vi "IDS Set Get Parameter.vi"(0 "IDS Notifier":refnum<notifier>, 5 "IDS Actions":T1, 7 "IDS Camera Ref":refnum<k24>, 11 "Error":errorcluster) -> (4 "IDS Notifier":refnum<notifier>, 15 "Error":errorcluster)   [LabVIEW 2021]
uses:
  IDS Controls/IDS Notifier Element.ctl
  IDS Controls/IDS Actions.ctl
  IDS Controls/IDS Parameters.ctl
  IDS Controls/IDS Parameter List.ctl
  IDS Controls/IDS ROI.ctl
  <vilib>/vision/Image Controls.llb/IMAQ Image.ctl
  C:/Users/Ries Lab/Documents/Microscope Control from Sheng Account/Microscope-Control/Device Library/Cameras/IDS/IDS LabView Examples/LabVIEW/ueye.NET/uEyeDotNet.dll
  IDS LabView Examples/LabVIEW/ueye.NET/uEyeDotNet.dll
panel:
  out "s32FactorNew":i32
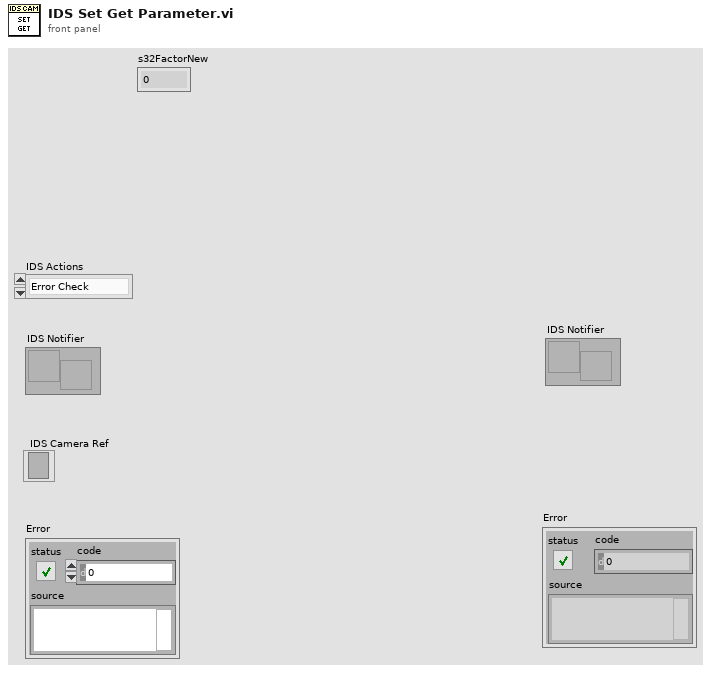
[diagram p1: front panel]
types:
  T1 = typedef "IDS Actions.ctl" = enum16{"Error Check", "Initialize", "Preview", "Record", "Abort", "Record Settings", "Set Parameter", "Get Parameter", "Set ROI", "Get ROI", "Status", "Quit"}
  T2 = typedef "IDS Notifier Element.ctl" = cluster{"IDS Actions":T1, "Received?":bool, "IDS Parameter":T3, "IDS ROI":T5, "Running?":bool, "File Path":path, "# of frames":u32, "Image Ref":T6, "Error":errorcluster, "Binning":i32}
  T3 = typedef "IDS Parameters.ctl" = cluster{"Parameter":T4, "Value":dbl}
  T4 = typedef "IDS Parameter List.ctl" = enum16{"Exposure Time (s)", "Binning", "Gain", "Gamma"}
  T5 = typedef "IDS ROI.ctl" = cluster{"H Offset":i32, "V Offset":i32, "H Width":i32, "V Width":i32}
  T6 = typedef "IMAQ Image.ctl" = refnum<image>
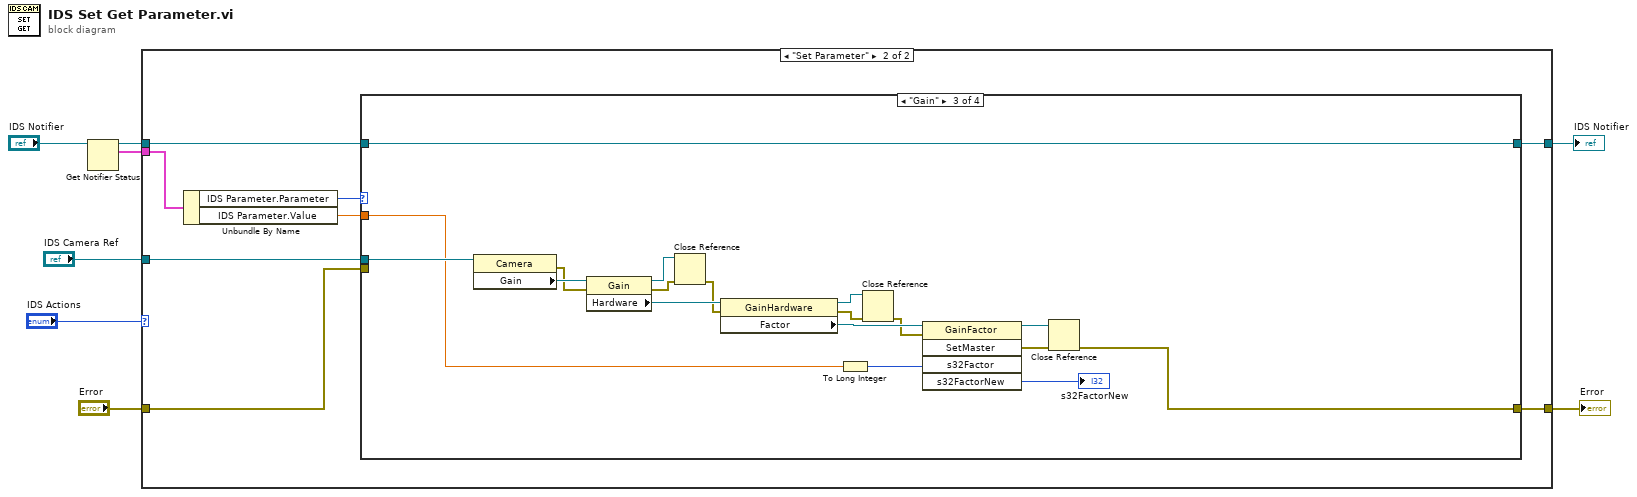
[diagram p0: block diagram]
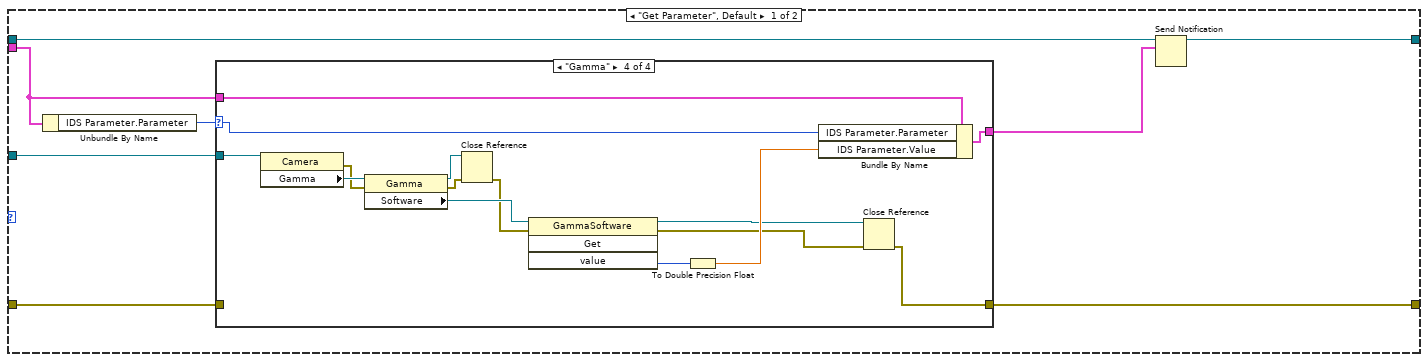
[diagram p2: hidden frame]
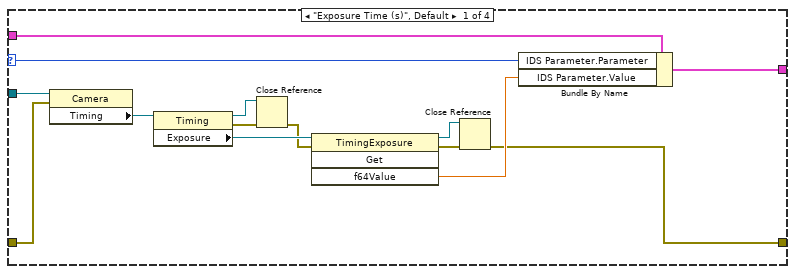
[diagram p3: hidden frame]
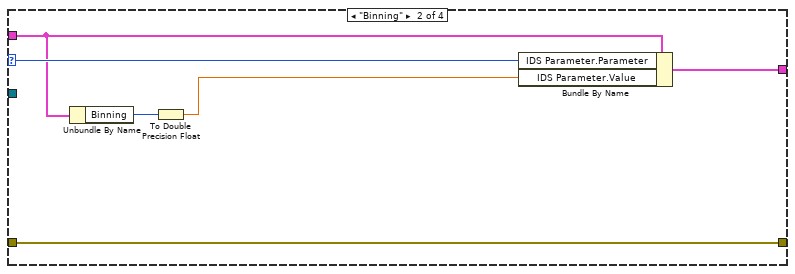
[diagram p4: hidden frame]
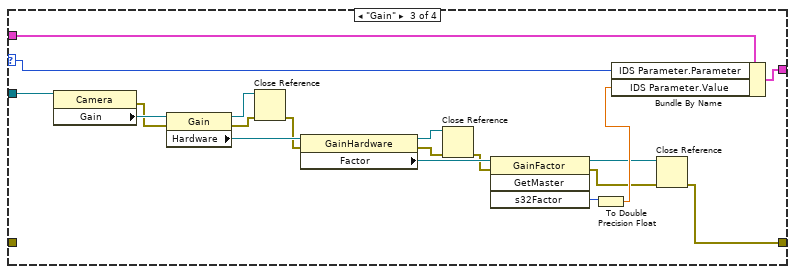
[diagram p5: hidden frame]
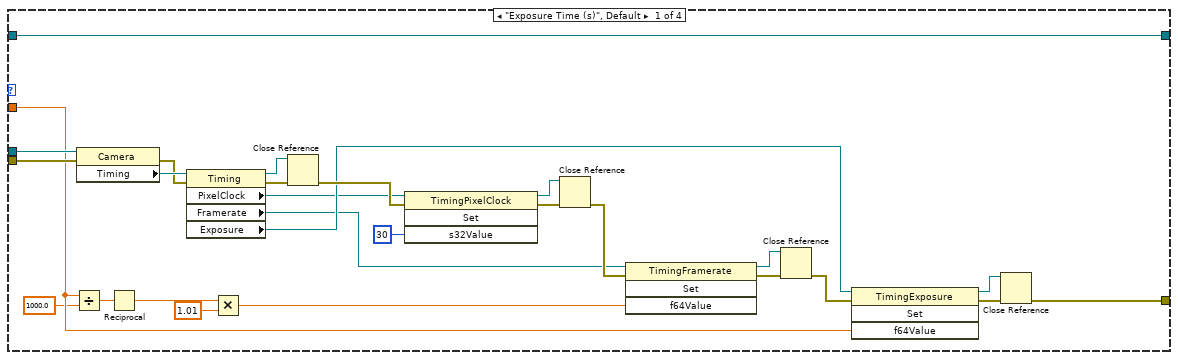
[diagram p6: hidden frame]
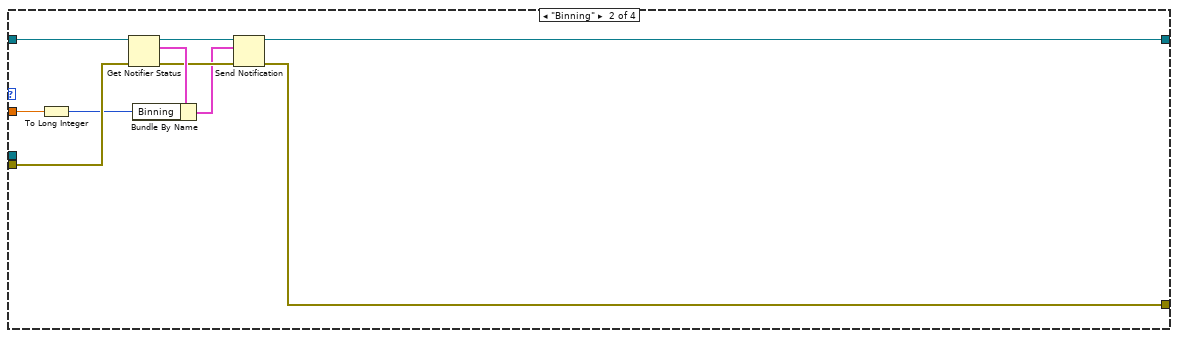
[diagram p7: hidden frame]
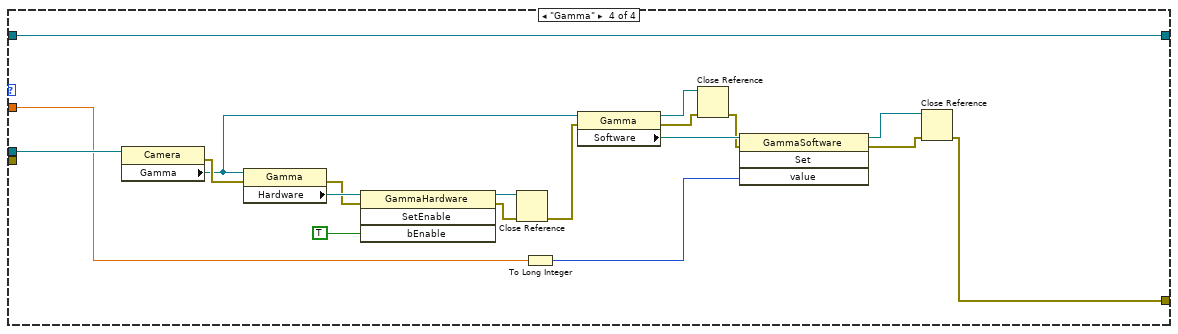
[diagram p8: hidden frame]
diagram:
  n1 = Get Notifier Status(notifier="IDS Notifier") -> (notifier out=w6:refnum<notifier>, current notification=w5:T2)  [unwired: 1 in, 3 out]
  n2 = case shown="\"Set Parameter\"" "IDS Actions" {
    tunnel: w6 -> [w11 w72]
    tunnel: w5 -> [w12 w78]
    tunnel: [w10 w71] -> w3
    tunnel: "IDS Camera Ref" -> [w13 w75]
    tunnel: "Error" -> [w15 w74]
    tunnel: [w14 w73] -> w1
    frame "Get Parameter", Default {
      n3 = Unbundle By Name(w12) -> ("IDS Parameter.Parameter"=w16:T4)
      n4 = case shown="\"Gamma\"" w16 {
        selector: w16 -> [w21 w36 w42 w63]
        tunnel: w15 -> [w18 w33 _ _]
        tunnel: [w17 w33 w37 w58] -> w14
        tunnel: w13 -> [w30 _ w45 w66]
        tunnel: w12 -> [w22 w34 w44 w65]
        tunnel: [w19 w35 w43 w64] -> w9
        frame "Exposure Time (s)", Default {
          n5 = property class="Camera"(reference=w30, error in=w18) -> ("Timing"=w29:refnum<k24>)  [unwired: 2 out]
          n6 = property class="Timing"(reference=w29) -> (reference out=w27:refnum<k24>, error out=w26:errorcluster, "Exposure"=w28:refnum<k24>)  [unwired: 1 in]
          n7 = Close Reference(reference=w27, error in (no error)=w26) -> (error out=w25:errorcluster)
          n8 = invoke class="TimingExposure" method="Get"(reference=w28, error in=w25) -> (reference out=w24:refnum<k24>, error out=w23:errorcluster, "f64Value"=w20:dbl)  [unwired: 2 in, 1 out]
          n9 = Close Reference(reference=w24, error in (no error)=w23) -> (error out=w17:errorcluster)
          n10 = Bundle By Name(cluster=w22, "IDS Parameter.Parameter"=w21, "IDS Parameter.Value"=w20) -> (w19:T2)
        }
        frame "Binning" {
          n11 = Unbundle By Name(w34) -> ("Binning"=w32:i32)
          n12 = To Double Precision Float(number=w32) -> (double precision float=w31:dbl)
          n13 = Bundle By Name(cluster=w34, "IDS Parameter.Parameter"=w36, "IDS Parameter.Value"=w31) -> (w35:T2)
        }
        frame "Gain" {
          n14 = property class="Camera"(reference=w45) -> (error out=w48:errorcluster, "Gain"=w55:refnum<k24>)  [unwired: 1 in, 1 out]
          n15 = property class="Gain"(reference=w55, error in=w48) -> (reference out=w51:refnum<k24>, error out=w50:errorcluster, "Hardware"=w54:refnum<k24>)
          n16 = Close Reference(reference=w51, error in (no error)=w50) -> (error out=w49:errorcluster)
          n17 = property class="GainHardware"(reference=w54, error in=w49) -> (reference out=w52:refnum<k24>, error out=w47:errorcluster, "Factor"=w53:refnum<k24>)
          n18 = Close Reference(reference=w52, error in (no error)=w47) -> (error out=w46:errorcluster)
          n19 = invoke class="GainFactor" method="GetMaster"(reference=w53, error in=w46) -> (reference out=w39:refnum<k24>, error out=w38:errorcluster, "s32Factor"=w41:i32)  [unwired: 2 in, 1 out]
          n20 = To Double Precision Float(number=w41) -> (double precision float=w40:dbl)
          n21 = Bundle By Name(cluster=w44, "IDS Parameter.Parameter"=w42, "IDS Parameter.Value"=w40) -> (w43:T2)
          n22 = Close Reference(reference=w39, error in (no error)=w38) -> (error out=w37:errorcluster)
        }
        frame "Gamma" {
          n23 = property class="Camera"(reference=w66) -> (error out=w67:errorcluster, "Gamma"=w70:refnum<k24>)  [unwired: 1 in, 1 out]
          n24 = property class="Gamma"(reference=w70, error in=w67) -> (reference out=w69:refnum<k24>, error out=w68:errorcluster, "Software"=w57:refnum<k24>)
          n25 = Close Reference(reference=w69, error in (no error)=w68) -> (error out=w56:errorcluster)
          n26 = invoke class="GammaSoftware" method="Get"(reference=w57, error in=w56) -> (reference out=w60:refnum<k24>, error out=w59:errorcluster, "value"=w62:i32)  [unwired: 2 in, 1 out]
          n27 = To Double Precision Float(number=w62) -> (double precision float=w61:dbl)
          n28 = Bundle By Name(cluster=w65, "IDS Parameter.Parameter"=w63, "IDS Parameter.Value"=w61) -> (w64:T2)
          n29 = Close Reference(reference=w60, error in (no error)=w59) -> (error out=w58:errorcluster)
        }
      }
      n30 = Send Notification(notification=w9, notifier=w11) -> (notifier out=w10:refnum<notifier>)  [unwired: 1 in, 1 out]
    }
    frame "Set Parameter" {
      n31 = Unbundle By Name(w78) -> ("IDS Parameter.Parameter"=w77:T4, "IDS Parameter.Value"=w76:dbl)
      n32 = case shown="\"Gain\"" w77 {
        tunnel: w76 -> [w83 w115 w128 w151]
        tunnel: w75 -> [w89 _ w133 w152]
        tunnel: w74 -> [w90 w111 _ _]
        tunnel: [w86 w106 w117 w148] -> w73
        tunnel: w72 -> [w79 w114 w120 w149]
        tunnel: [w79 w107 w120 w149] -> w71
        frame "Exposure Time (s)", Default {
          n33 = Divide(x=w83, y=1000.0) -> (x/y=w82:dbl)
          n34 = property class="Camera"(reference=w89, error in=w90) -> (error out=w92:errorcluster, "Timing"=w93:refnum<k24>)  [unwired: 1 out]
          n35 = Reciprocal(x=w82) -> (1/x=w85:dbl)
          n36 = property class="Timing"(reference=w93, error in=w92) -> (reference out=w97:refnum<k24>, error out=w98:errorcluster, "PixelClock"=w94:refnum<k24>, "Framerate"=w95:refnum<k24>, "Exposure"=w96:refnum<k24>)
          n37 = Multiply(x=w85, y=1.01) -> (x*y=w80:dbl)
          n38 = Close Reference(reference=w97, error in (no error)=w98) -> (error out=w99:errorcluster)
          n39 = invoke class="TimingPixelClock" method="Set"(reference=w94, error in=w99, "s32Value"=30 ("Pixelclock")) -> (reference out=w102:refnum<k24>, error out=w100:errorcluster)  [unwired: 1 in, 2 out]
          n40 = Close Reference(reference=w102, error in (no error)=w100) -> (error out=w101:errorcluster)
          n41 = invoke on="Methodenknoten" class="TimingFramerate" method="Set"(reference=w95, error in=w101, "f64Value"=w80) -> (reference out=w105:refnum<k24>, error out=w103:errorcluster)  [unwired: 1 in, 2 out]
          n42 = Close Reference(reference=w105, error in (no error)=w103) -> (error out=w104:errorcluster)
          n43 = invoke class="TimingExposure" method="Set"(reference=w96, error in=w104, "f64Value"=w83) -> (reference out=w87:refnum<k24>, error out=w88:errorcluster)  [unwired: 1 in, 2 out]
          n44 = Close Reference(reference=w87, error in (no error)=w88) -> (error out=w86:errorcluster)
        }
        frame "Binning" {
          n45 = To Long Integer(number=w115) -> (32bit integer=w109:i32)
          n46 = Get Notifier Status(notifier=w114, error in (no error)=w111) -> (notifier out=w112:refnum<notifier>, current notification=w113:T2, error out=w110:errorcluster)  [unwired: 2 out]
          n47 = Bundle By Name(cluster=w113, "Binning"=w109) -> (w108:T2)
          n48 = Send Notification(notification=w108, notifier=w112, error in (no error)=w110) -> (notifier out=w107:refnum<notifier>, error out=w106:errorcluster)
        }
        frame "Gain" {
          n49 = property class="Camera"(reference=w133) -> (error out=w123:errorcluster, "Gain"=w132:refnum<k24>)  [unwired: 1 in, 1 out]
          n50 = property class="Gain"(reference=w132, error in=w123) -> (reference out=w126:refnum<k24>, error out=w125:errorcluster, "Hardware"=w131:refnum<k24>)
          n51 = Close Reference(reference=w126, error in (no error)=w125) -> (error out=w124:errorcluster)
          n52 = property class="GainHardware"(reference=w131, error in=w124) -> (reference out=w127:refnum<k24>, error out=w122:errorcluster, "Factor"=w130:refnum<k24>)
          n53 = To Long Integer(number=w128) -> (32bit integer=w129:i32)
          n54 = Close Reference(reference=w127, error in (no error)=w122) -> (error out=w121:errorcluster)
          n55 = invoke class="GainFactor" method="SetMaster"(reference=w130, error in=w121, "s32Factor"=w129) -> (reference out=w118:refnum<k24>, error out=w119:errorcluster, "s32FactorNew"=→"s32FactorNew":i32)  [unwired: 2 in, 2 out]
          n56 = Close Reference(reference=w118, error in (no error)=w119) -> (error out=w117:errorcluster)
        }
        frame "Gamma" {
          n57 = property class="Camera"(reference=w152) -> (error out=w150:errorcluster, "Gamma"=w144:refnum<k24>)  [unwired: 1 in, 1 out]
          n58 = property class="Gamma"(reference=w144, error in=w150) -> (error out=w145:errorcluster, "Hardware"=w147:refnum<k24>)  [unwired: 1 out]
          n59 = invoke class="GammaHardware" method="SetEnable"(reference=w147, error in=w145, "bEnable"=TRUE) -> (reference out=w142:refnum<k24>, error out=w141:errorcluster)  [unwired: 1 in, 2 out]
          n60 = Close Reference(reference=w142, error in (no error)=w141) -> (error out=w140:errorcluster)
          n61 = To Long Integer(number=w151) -> (32bit integer=w136:i32)
          n62 = property class="Gamma"(reference=w144, error in=w140) -> (reference out=w139:refnum<k24>, error out=w138:errorcluster, "Software"=w143:refnum<k24>)
          n63 = Close Reference(reference=w139, error in (no error)=w138) -> (error out=w137:errorcluster)
          n64 = invoke class="GammaSoftware" method="Set"(reference=w143, error in=w137, "value"=w136) -> (reference out=w135:refnum<k24>, error out=w134:errorcluster)  [unwired: 1 in, 2 out]
          n65 = Close Reference(reference=w135, error in (no error)=w134) -> (error out=w148:errorcluster)
        }
      }
    }
  }
  "IDS Notifier" <- w3
  "Error" <- w1
